vi "UnscentedKalmanFilter_Correct_OnlyUYR.vi"(4 "H_ExtraData":variant, 6 "H":T1, 7 "Rows":i32, 8 "R":T2, 9 "Y":T2, 10 "U":T2, 11 "in UnscentedKalmanFiilter":T3) -> (0 "Error":bool, 3 "out UnscentedKalmanFiilter":T3)   [LabVIEW 2019, in "Trajectory_Library.lvlib"]
doc: "Correct the state estimate x-hat using the measurements in y.\n \nThis is useful for when the measurements available during a timestep's Correct() call vary.\nThe h(x, u) passed to the constructor is used if one is not provided (the two-argument version\nof this function).\n \nInputs:\n - inUnscentedKalmanFilter -- filter data cluster\n - rows -- Number of rows in y.\n - u -- Same control input used in the predict step.\n - y -- Measurement vector.\n - R -- Measurement noise covariance matrix (continuous-time).\n - H_Func -- A vector-valued function of x and u that returns the measurement vector.\n - H_ExtraData -- A variant containing extra data used by the H function. The contents are specific to each different H function.\n\nOutputs:\n - outUnscentedKalmanFilter -- updated filter data cluster\n - Error -- If TRUE, an error occured."
uses:
  Trajectory_Library.lvlib
  <vilib>/Analysis/Matrix/Datatypes/RealMatrix.ctl
  <vilib>/Analysis/Matrix/NI_Matrix.lvlib
  TypeDef/MERWE_SCALED_SIGMA_PTS.ctl
  TypeDef/UNSCENTED_KALMAN_FILTER.ctl
  TypeDef/CALLBACK_FUNC_TYPE.ctl
panel:
  # "<Inputs, 1>"
  # "<Rows, 1>"
  # "<Rows, Rows>"
  # "State Estimate <Statess,1>"
  # "<States, States>"
  # "<States, ?>"
  # "<Statess,  States>"
  # "<Outputs, Outputs>"
  # "<?, 1>"
  # "<?, 1>"
  # "State Estimate <Statess,1>"
  # "<States, States>"
  # "<States, ?>"
  # "<Statess,  States>"
  # "<Outputs, Outputs>"
  # "<?, 1>"
  # "<?, 1>"
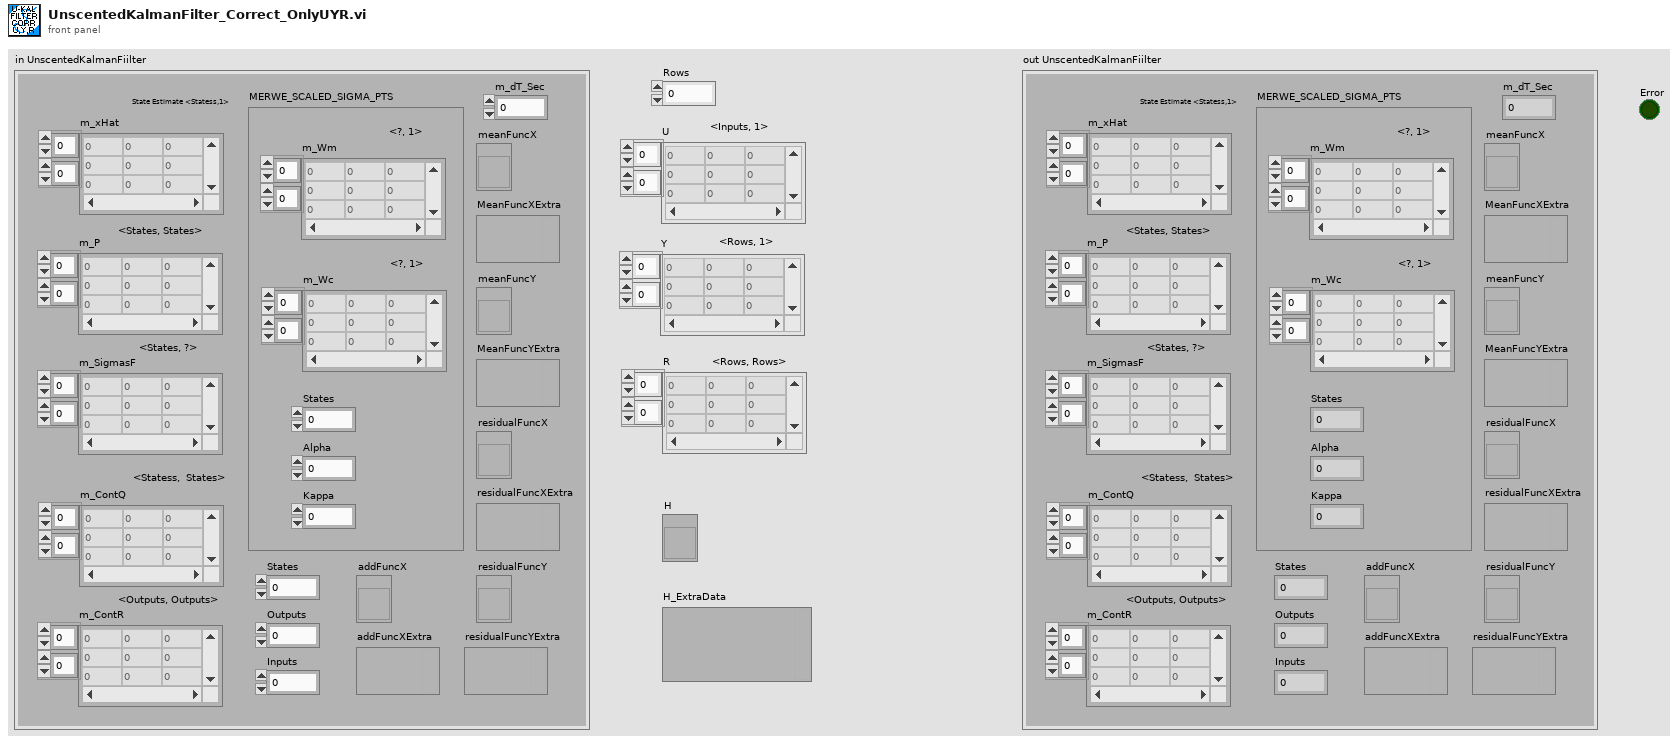
[diagram p1: front panel]
types:
  T1 = typedef "Trajectory_Library.lvlib/CALLBACK_FUNC_TYPE.ctl" = refnum<vi>
  T2 = typedef "NI_Matrix.lvlib/RealMatrix.ctl" = dbl[][]
  T3 = typedef "Trajectory_Library.lvlib/UNSCENTED_KALMAN_FILTER.ctl" = cluster{"m_P":T2, "m_xHat":T2, "States":i32, "Outputs":i32, "m_ContR":T2, "m_ContQ":T2, "m_SigmasF":T2, "m_dT_Sec":dbl, "MERWE_SCALED_SIGMA_PTS":T4, "meanFuncX":T1, "meanFuncY":T1, "residualFuncX":T1, "residualFuncY":T1, "addFuncX":T1, "addFuncXExtra":variant, "residualFuncYExtra":variant, "residualFuncXExtra":variant, "MeanFuncYExtra":variant, "MeanFuncXExtra":variant, "Inputs":i32}
  T4 = typedef "Trajectory_Library.lvlib/MERWE_SCALED_SIGMA_PTS.ctl" = cluster{"m_Wm":T2, "States":i32, "Alpha":dbl, "m_Wc":T2, "Kappa":i32}
  T5 = typedef "WPILib_Math.lvlib/UNSCENTED_KALMAN_CORRECT_FUNC_GROUP.ctl" = cluster{"H_Func":T6, "meanFuncY":T6, "residualFuncY":T6, "residualFuncX":T6, "addFuncX":T6, "H_FuncExtra":variant, "MeanFuncYExtra":variant, "residualFuncYExtra":variant, "residualFuncXExtra":variant, "addFuncXExtra":variant}
  T6 = typedef "WPILib_Math.lvlib/CALLBACK_FUNC_TYPE.ctl" = refnum<vi>
  T7 = typedef "WPILib_Math.lvlib/UNSCENTED_KALMAN_FILTER.ctl" = cluster{"m_P":T2, "m_xHat":T2, "States":i32, "Outputs":i32, "m_ContR":T2, "m_ContQ":T2, "m_SigmasF":T2, "m_dT_Sec":dbl, "MERWE_SCALED_SIGMA_PTS":T8, "meanFuncX":T6, "meanFuncY":T6, "residualFuncX":T6, "residualFuncY":T6, "addFuncX":T6, "addFuncXExtra":variant, "residualFuncYExtra":variant, "residualFuncXExtra":variant, "MeanFuncYExtra":variant, "MeanFuncXExtra":variant, "Inputs":i32}
  T8 = typedef "WPILib_Math.lvlib/MERWE_SCALED_SIGMA_PTS.ctl" = cluster{"m_Wm":T2, "States":i32, "Alpha":dbl, "m_Wc":T2, "Kappa":i32}
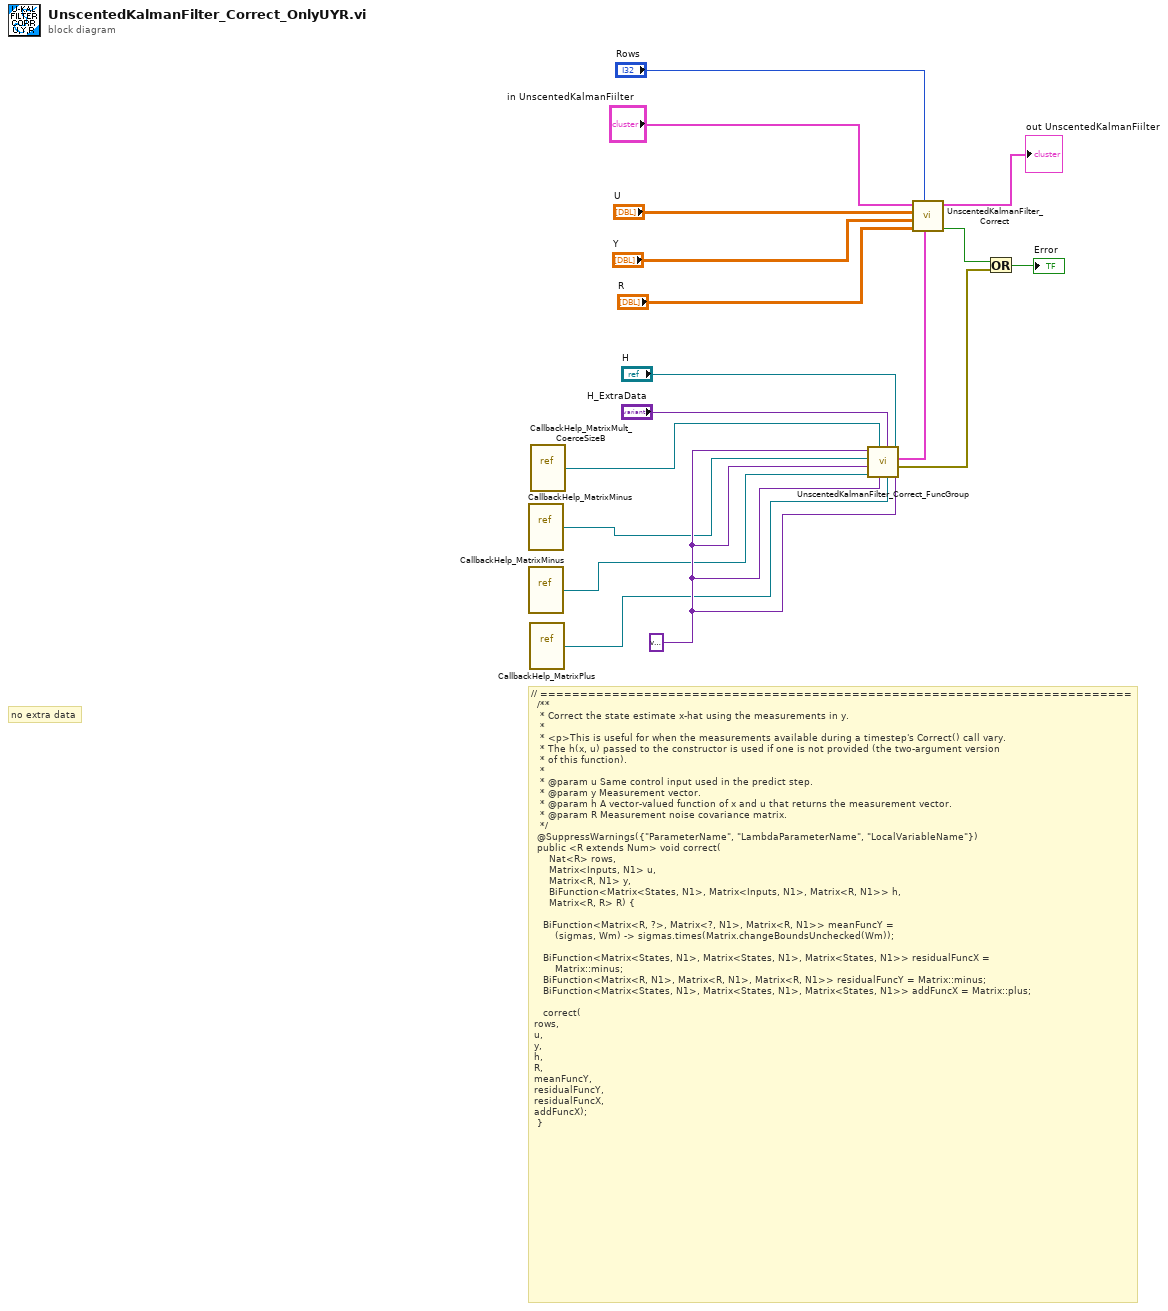
[diagram p0: block diagram]
diagram:
  w5 = variant ("addFuncXExtra")
  # "no extra data"
  # "// ==========================================================================\n  /**\n   * Correct the state estimate x-hat using the measurements in y.\n   *\n   * <p>This is useful for when the measurements available during a timestep's Correct() call vary.\n   * The h(x, u) passed to the constructor is used if one is not provided (the two-argument version\n   * of this function).\n   *\n   * @param u Same control input used in the predict step.\n   * @param y Measurement vector.\n   * @param h A vector-valued function of x and u that returns the measurement vector.\n   * @param R Measurement noise covariance matrix.\n   */\n  @SuppressWarnings({\"ParameterName\", \"LambdaParameterName\", \"LocalVariableName\"})\n  public <R extends Num> void correct(\n      Nat<R> rows,\n      Matrix<Inputs, N1> u,\n      Matrix<R, N1> y,\n      BiFunction<Matrix<States, N1>, Matrix<Inputs, N1>, Matrix<R, N1>> h,\n      Matrix<R, R> R) {\n\n    BiFunction<Matrix<R, ?>, Matrix<?, N1>, Matrix<R, N1>> meanFuncY =\n        (sigmas, Wm) -> sigmas.times(Matrix.changeBoundsUnchecked(Wm));\n    \n    BiFunction<Matrix<States, N1>, Matrix<States, N1>, Matrix<States, N1>> residualFuncX =\n        Matrix::minus;\n    BiFunction<Matrix<R, N1>, Matrix<R, N1>, Matrix<R, N1>> residualFuncY = Matrix::minus;\n    BiFunction<Matrix<States, N1>, Matrix<States, N1>, Matrix<States, N1>> addFuncX = Matrix::plus;\n    \n    correct(\n\trows, \n\tu, \n\ty, \n\th, \n\tR, \n\tmeanFuncY, \n\tresidualFuncY, \n\tresidualFuncX, \n\taddFuncX);\n  }"
  n1 = vi-ref "CallbackHelp_MatrixMinus.vi"() -> (w2:refnum<vi>)
  n2 = vi-ref "CallbackHelp_MatrixMinus.vi"() -> (w3:refnum<vi>)
  n3 = vi-ref "CallbackHelp_MatrixPlus.vi"() -> (w4:refnum<vi>)
  n4 = vi-ref "CallbackHelp_MatrixMult_CoerceSizeB.vi"() -> (w1:refnum<vi>)
  n5 = call "UnscentedKalmanFilter_Correct_FuncGroup.vi"("addFuncXExtra"=w5, "H_Func"="H", "AddFuncX"=w4, "H_FuncExtra"="H_ExtraData", "residualFuncXExtra"=w5, "MeanFuncY"=w1, "ResidualFuncX"=w3, "residualFuncYExtra"=w5, "ResidualFuncY"=w2, "MeanFuncYExtra"=w5) -> ("Error"=w6:errorcluster, "UNSCENTED_KALMAN_CORRECT_FUNC_GROUP"=w12:T5)
  n6 = call "UnscentedKalmanFilter_Correct.vi"("UNSCENTED_KALMAN_CORRECT_FUNC_GROUP"=w12, "Rows"="Rows", "R"="R", "Y"="Y", "U"="U", "in UnscentedKalmanFiilter"="in UnscentedKalmanFiilter") -> ("Error"=w7:bool, "out UnscentedKalmanFiilter"=→"out UnscentedKalmanFiilter":T7)  [unwired: 4 in]
  n7 = Or(x=w7, y=w6) -> (x .or. y?=→"Error":bool)
